vi "validate Max Value.vi"(9 "Max Index":i32[](array[numeric]), 11 "Trace Values":T1 {"Frequency" format="%#_6p"}) -> (1 "Frequency":dbl[](array[numeric]), 2 "isExceed?":bool[](array[boolean]), 3 "Amplitude":dbl[](array[numeric]))   [LabVIEW 2023, in "Instrument Manager.lvclass"]
uses:
  Instrument Manager.lvclass
  Module/Spectrum Analyzer/TYPE DEFINITION/TYPE Trace Value Array.ctl
  Module/Spectrum Analyzer/Spectrum Analyzer.lvlib
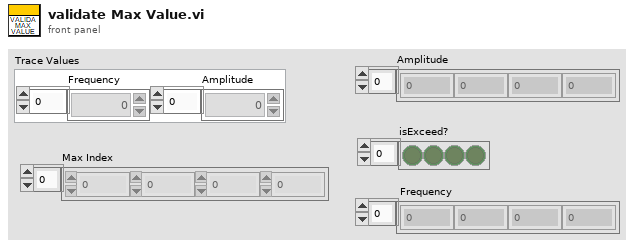
[diagram p1: front panel]
types:
  T1 = typedef "Spectrum Analyzer.lvlib/TYPE Trace Value Array.ctl" = cluster{"Frequency":dbl[], "Amplitude":dbl[]}
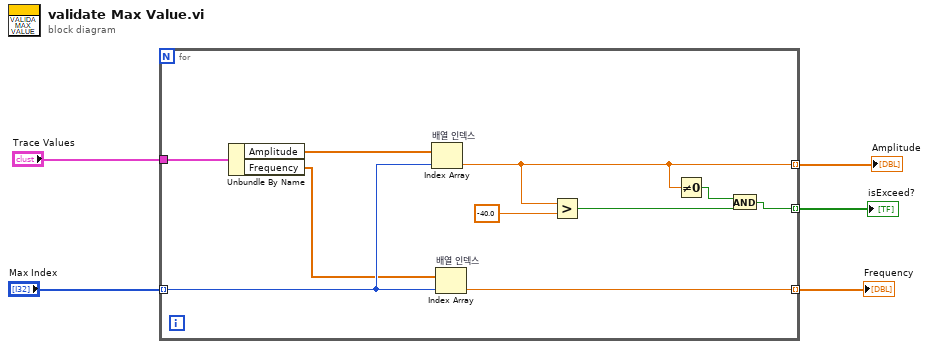
[diagram p0: block diagram]
diagram:
  n1 = for {
    tunnel: "Max Index" -> [w12] mode=indexing
    tunnel: "Trace Values" -> [w15]
    tunnel: [w9] -> w3 mode=indexing
    tunnel: [w6] -> w2 mode=indexing
    tunnel: [w10] -> w1 mode=indexing
    n2 = Unbundle By Name(w15) -> ("Amplitude"=w14:dbl[], "Frequency"=w11:dbl[])
    n3 = Index Array "배열 인덱스"(array=w14, index=w12) -> (element=w9:dbl)
    n4 = Index Array "배열 인덱스"(array=w11, index=w12) -> (element=w10:dbl)
    n5 = Greater?(x=w9, y=-40.0) -> (0:w7:bool)
    n6 = Not Equal To 0?(x=w9) -> (x != 0?=w8:bool)
    n7 = And(x=w8, y=w7) -> (x .and. y?=w6:bool)
  }
  "Amplitude" <- w3
  "isExceed?" <- w2
  "Frequency" <- w1
